vi "RDV-writePlotSettings.vi"(8 "error in (no error)":errorcluster, 10 "Plot Settings":T1={"common name to remove"="", "Max Size"=18}, 11 "RDV-Reflection_Data_viewer in":refnum<class "RDV-Reflection_Data_viewer.lvclass">) -> (0 "error out":errorcluster, 3 "RDV-Reflection_Data_viewer out":refnum<class "RDV-Reflection_Data_viewer.lvclass">)   [LabVIEW 2020, in "RDV-Reflection_Data_viewer.lvclass"]
doc: "Writes the plot settings (common name to remove, max size) into the viewer object."
uses:
  RDV-Reflection_Data_viewer.lvclass
  RDV-PLOT_SETTINGS.ctl
  RDV-Reflection_Data_viewer.lvclass/RDV-Reflection_Data_viewer.ctl
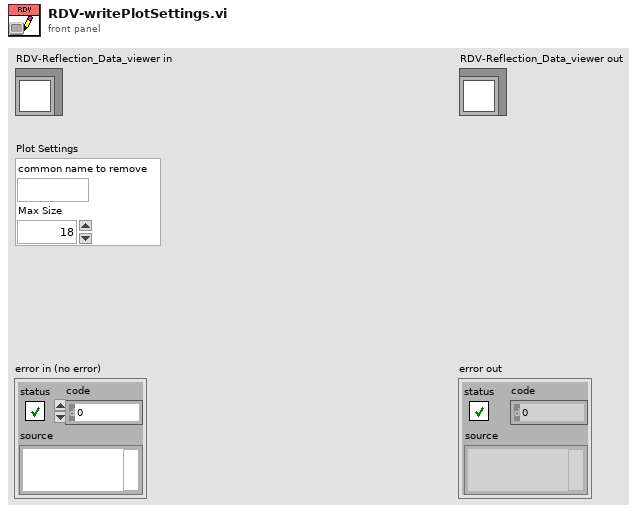
[diagram p1: front panel]
types:
  T1 = typedef "RDV-Reflection_Data_viewer.lvclass/RDV-PLOT_SETTINGS.ctl" = cluster{"common name to remove":string, "Max Size":i32}
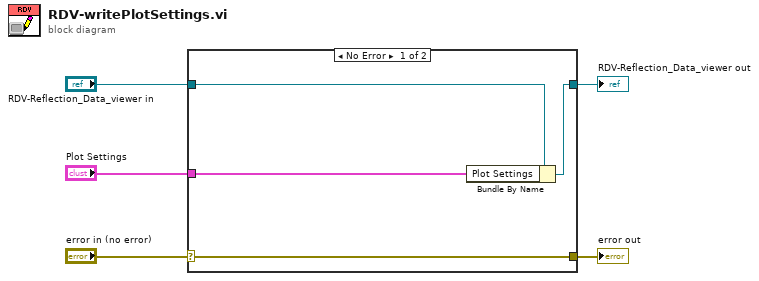
[diagram p0: block diagram]
diagram:
  n1 = case shown="No Error" "error in (no error)" {
    selector: "error in (no error)" -> [w9 w10]
    tunnel: [w9 w10] -> w4
    tunnel: [w7 w11] -> w2
    tunnel: "RDV-Reflection_Data_viewer in" -> [w8 w11]
    tunnel: "Plot Settings" -> [w6 _]
    frame No Error {
      n2 = Bundle By Name(cluster=w8, "Plot Settings"=w6) -> (w7:refnum<class "RDV-Reflection_Data_viewer.lvclass">)
    }
    frame Error {
    }
  }
  "error out" <- w4
  "RDV-Reflection_Data_viewer out" <- w2
